vi "close sys config device.vi"(8 "error in":errorcluster, 11 "controller in":refnum<class "Controller.lvclass">) -> (0 "error out":errorcluster, 3 "controller out":refnum<class "Controller.lvclass">)   [LabVIEW 2014, in "SMI.lvlib" / "SysCfg Device.lvclass"]
uses:
  SysCfg Device.lvclass
  Controller/Controller.lvclass
  <vilib>/nisyscfg/Close (System).vi
  <vilib>/nisyscfg/Close (Hardware).vi
  Controller/read system hardware ref.vi
  read system session.vi
  <vilib>/nisyscfg/nisyscfg.lvlib
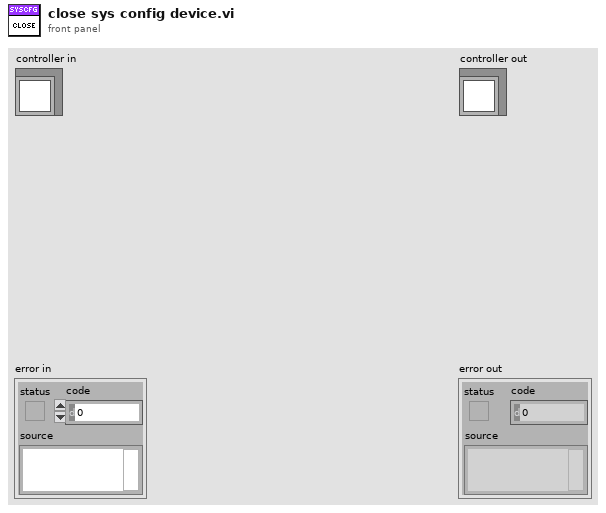
[diagram p1: front panel]
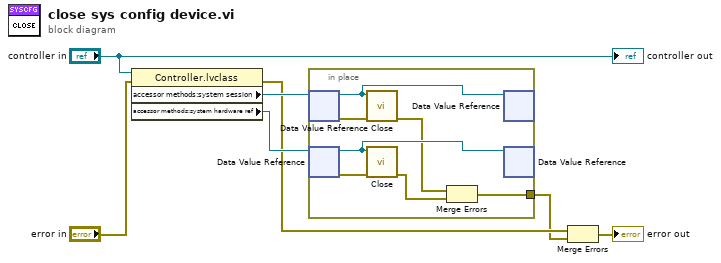
[diagram p0: block diagram]
diagram:
  n1 = property class="Controller.lvclass"(reference="controller in", error in="error in") -> (error out=w3:errorcluster, "accessor methods:system session"=w5:refnum<data-value>, "accessor methods:system hardware ref"=w4:refnum<data-value>)  [unwired: 1 out]
  n2 = in-place {
    in-place-border: [w8] -> w2
    n3 = in-place-dvr #1(w5) -> (w14:refnum<k21>, w12:errorcluster)
    n4 = in-place-dvr #2(w4) -> (w13:refnum<k20>, w11:errorcluster)
    n5 = call-poly <vilib>:"Close.vi"("error in (no error)"=w12, "Session in"=w14) -> ("error out"=w10:errorcluster)  [unwired: 9 in]
    n6 = call-poly <vilib>:"Close.vi"("error in (no error)"=w11, "Resource in"=w13) -> ("error out"=w9:errorcluster)  [unwired: 9 in]
    n7 = Merge Errors(w10, w9) -> (w8:errorcluster)
    n8 = in-place-dvr #1(w14) -> ()  [unwired: 2 out]
    n9 = in-place-dvr #2(w13) -> ()  [unwired: 2 out]
  }
  n10 = Merge Errors(w3, w2) -> (→"error out":errorcluster)
  "controller out" <- "controller in"
